vi "Fix Velocities from Joysticks.vi"(10 "Axes":dbl[](array[numeric]), 11 "Deadband":cluster{"value":dbl, "value":dbl, "value":dbl}) -> (1 "Sending Input?":bool, 2 "Adjusted Robot Velocities":T1)   [LabVIEW 2027]
uses:
  swerve-template/Type Definitions/Data/Robot Velocities.ctl
  3ad3cf1c-8863-4f6c-a2e6-a00d4e593ecd.vi
  <vilib>/MRC/Types/XBox Axes Index.ctl
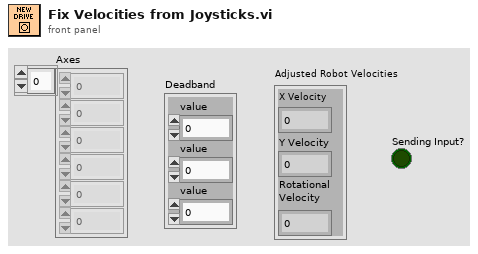
[diagram p1: front panel]
types:
  T1 = typedef "Robot Velocities.ctl" = cluster{"X Velocity":dbl, "Y Velocity":dbl, "Rotational \nVelocity":dbl}
  T2 = typedef "XBox Axes Index.ctl" = enum16{"Left X", "Left Y", "Left Trigger", "Right Trigger", "Right X", "Right Y"}
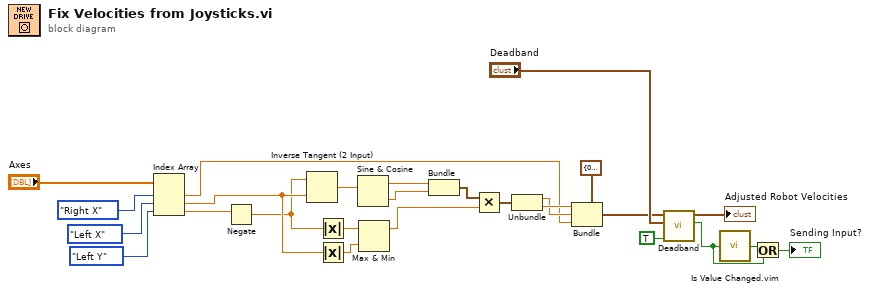
[diagram p0: block diagram]
diagram:
  n1 = Index Array(array="Axes", index #1=XBox_Axes_Index."Right X" ("XBox Axes"), index #2=XBox_Axes_Index."Left X" ("XBox Axes"), index #3=XBox_Axes_Index."Left Y" ("XBox Axes")) -> (element #1=w4:dbl, element #2=w21:dbl, element #3=w17:dbl)
  n2 = Negate(x=w17) -> (-x=w16:dbl)
  n3 = Inverse Tangent (2 Input)(1:w21, 2:w16) -> (0:w13:dbl)
  n4 = Absolute Value(x=w16) -> (abs(x)=w10:dbl)
  n5 = Absolute Value(x=w21) -> (abs(x)=w9:dbl)
  n6 = Sine & Cosine(0:w13) -> (1:w12:dbl, 2:w11:dbl)
  n7 = Max & Min(x=w10, y=w9) -> (max(x,y)=w7:dbl)  [unwired: 1 out]
  n8 = Bundle(w12, w11) -> (w8:cluster{dbl, dbl})  [unwired: 1 in]
  n9 = Multiply(x=w8, y=w7) -> (x*y=w6:cluster{dbl, dbl})
  n10 = Unbundle(w6) -> (w5:dbl, w14:dbl)
  n11 = Bundle(cluster=cluster{dbl, dbl, "upper limit":dbl} {0.0, 0.0, "upper limit"=0.0}, w14, w5, "upper limit"=w4) -> (w23:cluster{dbl, dbl, "upper limit":dbl})
  n12 = call "Deadband.vi"("Rescaling On?"=TRUE, "Deadband Info"="Deadband", "Robot Velocities"=w23) -> ("Sending Input?"=w19:bool, "Adjusted Robot Velocities"=→"Adjusted Robot Velocities":T1)  [unwired: 7 in]
  n13 = call "Is Value Changed.vim"("value"=w19) -> ("changed or first call?"=w20:bool)
  n14 = Or(x=w20, y=w19) -> (x .or. y?=→"Sending Input?":bool)
